vi "Default Tool Arguments.vi"(8 "error in":errorcluster, 11 "message json":string) -> (0 "error out":errorcluster, 3 "message json out":string)   [LabVIEW 2020, in "MCP Server.lvlib"]
doc: "arguments is optional in tools/call. If the request has no arguments member, this VI adds an empty one (\"arguments\": {}), so the tool is called with the default values of its inputs.\n\nA request that has an arguments member is passed through unchanged, whatever its value is."
uses:
  MCP Server.lvlib
  <vilib>/JDP Science/JSONtext/Next JSON Value.vi
  <vilib>/JDP Science/JSONtext/String Subset.vi
  <vilib>/JDP Science/JSONtext/Parsing/Advance past next JSON Value (inlined COPY).vi
  <vilib>/JDP Science/JSONtext/Parsing/Advance past whitespace.vi
  <vilib>/JDP Science/JSONtext/Parsing/Advance past String.vi
  <vilib>/JDP Science/JSONtext/Parsing/Advance past Number.vi
  <vilib>/JDP Science/JSONtext/Parsing/Advance past Line Ending.vi
  <vilib>/JDP Science/JSONtext/Parsing/Parse Full Path or Item Name.vi
  <vilib>/JDP Science/JSONtext/Parsing/Advance past Array.vi
  <vilib>/JDP Science/JSONtext/Parsing/Advance past Object.vi
  <vilib>/JDP Science/JSONtext/support/Error Cluster From Code.vi
  <vilib>/JDP Science/JSONtext/Offset/Find Item Locations by Path.vi
  <vilib>/JDP Science/JSONtext/JSONtext.lvlib
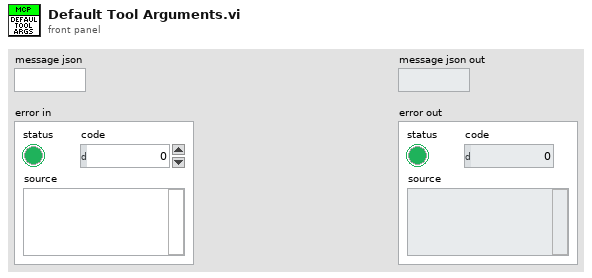
[diagram p1: front panel]
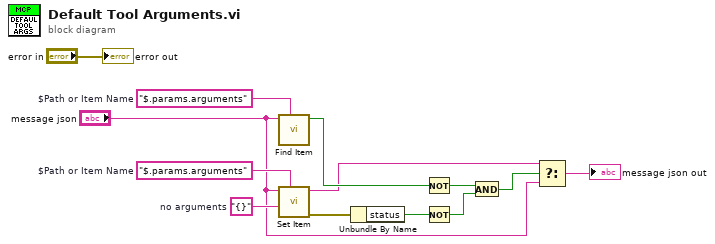
[diagram p0: block diagram]
diagram:
  w11 = "{}"  # no arguments
  w12 = "$.params.arguments"  # $Path or Item Name
  w13 = "$.params.arguments"  # $Path or Item Name
  n1 = call <vilib>:"Find Item.vi"("$Path or Item Name"=w13, "JSON"="message json") -> ("Found"=w10:bool)  [unwired: 6 in, 3 out]
  n2 = call <vilib>:"Set Item.vi"("$Path or Item Name"=w12, "JSON to Insert"=w11, "JSON"="message json") -> ("error out"=w9:errorcluster, "<JSON>"=w5:string)  [unwired: 5 in, 1 out]
  n3 = Unbundle By Name(w9) -> ("status"=w8:bool)
  n4 = Not(x=w10) -> (.not. x?=w7:bool)
  n5 = Not(x=w8) -> (.not. x?=w6:bool)
  n6 = And(x=w7, y=w6) -> (x .and. y?=w4:bool)
  n7 = Select(t=w5, s=w4, f="message json") -> (s? t:f=→"message json out":string)
  "error out" <- "error in"
